vi "VIH ProjFile - XML - Get Child Elements.vi"(8 "error in":errorcluster, 10 "Tag Name":string, 11 "XML Parent Item":refnum<k20>) -> (0 "error out":errorcluster, 2 "Array of Elements":refnum<k20>[](array[refnum]), 3 "dup XML Parent Item":refnum<k20>)   [LabVIEW 2014]
doc: "::: VI Helpeks :::\nCopyright (c) 2000-2026 Konstantin Shifershteyn. All rights reserved."
uses:
  <vilib>/xml/Close Reference(Node).vi
  <resource>/objmgr/DOMUserDefRef.rc
  <vilib>/xml/NI_XML.lvlib
panel:
  # "VI Helpeks\nCopyright (c) 2012-2026 Konstantin Shifershteyn"
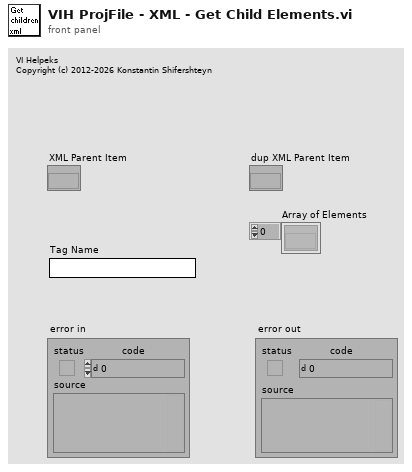
[diagram p1: front panel]
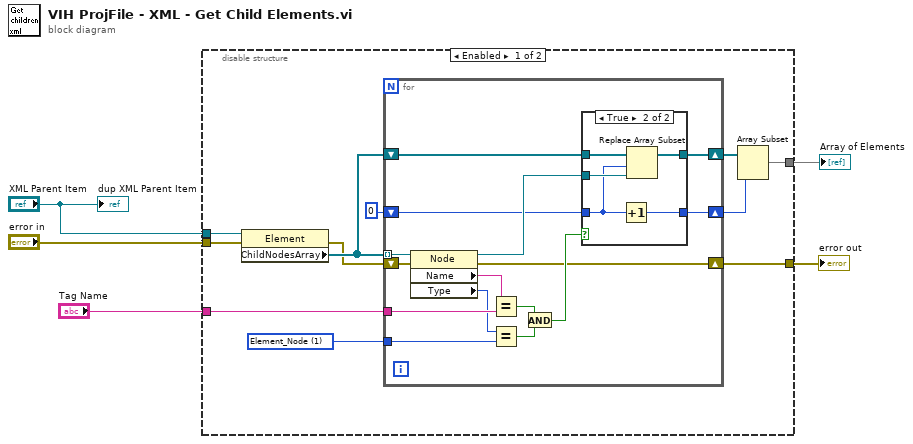
[diagram p0: block diagram]
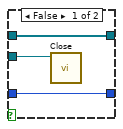
[diagram p2: hidden frame]
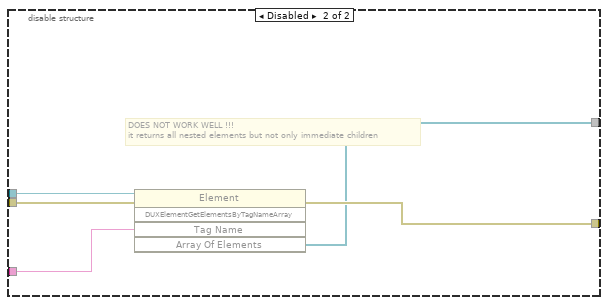
[diagram p3: hidden frame]
diagram:
  n1 = disable-structure shown="Enabled" {
    disable-tunnel: "XML Parent Item" -> [w16 w42]
    disable-tunnel: "error in" -> [w15 w44]
    disable-tunnel: "Tag Name" -> [w14 w41]
    disable-tunnel: [w7 w40] -> w2
    disable-tunnel: [w6 w43] -> w1
    frame Enabled {
      w13 = 1 items=["Element_Node"=1, "Attribute_Node"=2, "Text_Node"=3, "CDATASection_Node"=4, "EntityReference_Node"=5, "Entity_Node"=6, "ProcessingInstruction_Node"=7, "Comment_Node"=8, "Document_Node"=9, "DocumentType_Node"=10, "DocumentFragment_Node"=11, "Notation_Node"=12] ("Node Type")
      n2 = property class="Element"(reference=w16, error in=w15) -> (error out=w10:errorcluster, "ChildNodesArray"=w12:refnum<k20>[])  [unwired: 1 out]
      n3 = for {
        tunnel: w12 -> [w31] mode=indexing
        shift-right: [w21] -> w9
        shift-left: w12 -> [w23]
        tunnel: w14 -> [w29]
        tunnel: w13 -> [w27]
        shift-right: [w19] -> w8
        shift-left: 0 -> [w20]
        shift-right: [w17] -> w6
        shift-left: w10 -> [w18]
        n4 = property class="Node"(reference=w31, error in=w18) -> (reference out=w22:refnum<k20>, error out=w17:errorcluster, "Name"=w30:string, "Type"=w28:i32)
        n5 = Equal?(x=w30, y=w29) -> (x = y?=w26:bool)
        n6 = Equal?(x=w28, y=w27) -> (x = y?=w25:bool)
        n7 = And(x=w26, y=w25) -> (x .and. y?=w24:bool)
        n8 = case shown="True" w24 {
          tunnel: w23 -> [w34 w39]
          tunnel: w22 -> [w32 w37]
          tunnel: [w34 w38] -> w21
          tunnel: w20 -> [w33 w36]
          tunnel: [w33 w35] -> w19
          frame False {
            n9 = call-poly <vilib>:"Close.vi"("node"=w32) -> ()  [unwired: 8 in, 1 out]
          }
          frame True {
            n10 = Increment(x=w36) -> (x+1=w35:i32)
            n11 = Replace Array Subset(array=w39, new element=w37, index=w36) -> (w38:refnum<k20>[])
          }
        }
      }
      n12 = Array Subset(array=w9, length=w8) -> (w7:refnum<k20>[])  [unwired: 1 in]
    }
    frame Disabled {
      # "DOES NOT WORK WELL !!!\nit returns all nested elements but not only immediate children"
      n13 = invoke class="Element" method="DUXElementGetElementsByTagNameArray"(reference=w42, error in=w44, "Tag Name"=w41) -> (error out=w43:errorcluster, "Array Of Elements"=w40:refnum<k20>[])  [unwired: 2 in, 3 out]
    }
  }
  "error out" <- w1
  "Array of Elements" <- w2
  "dup XML Parent Item" <- "XML Parent Item"
